vi "GetConnectionStatus.vi"(8 "error in (no error)":errorcluster, 11 "object in":refnum<class "DIO_Channel.lvclass">) -> (0 "error out":errorcluster, 2 "Connected?":bool, 3 "object out":refnum<class "DIO_Channel.lvclass">)   [LabVIEW 2021, in "Simulator-Channel.lvlib" / "DIO_Channel.lvclass"]
uses:
  DIO_Channel.lvclass
  <vilib>/ActorFramework/Message Enqueuer/Message Enqueuer.lvclass
  DIO_Channel.lvclass/DIO_Channel.ctl
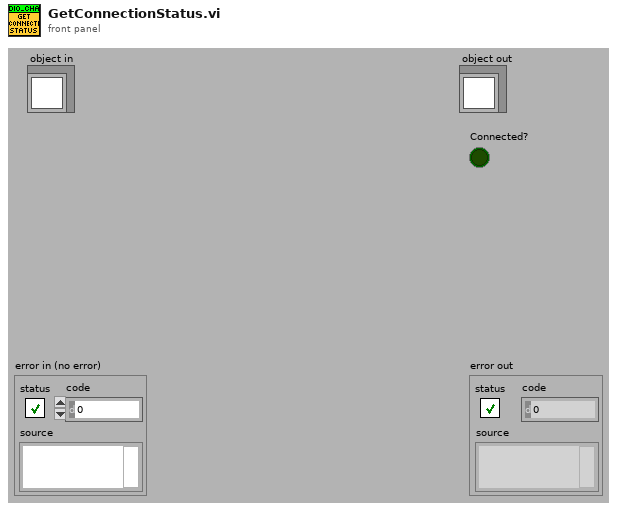
[diagram p1: front panel]
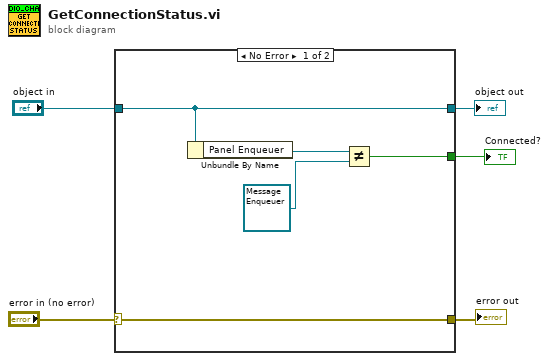
[diagram p0: block diagram]
diagram:
  n1 = case shown="No Error" "error in (no error)" {
    selector: "error in (no error)" -> [w10 w12]
    tunnel: [w10 w12] -> w4
    tunnel: [w9 w11] -> w2
    tunnel: "object in" -> [w9 w11]
    tunnel: [w6 _] -> w1
    frame No Error {
      n2 = Unbundle By Name(w9) -> ("Panel Enqueuer"=w8:refnum<class "Message Enqueuer.lvclass">)
      n3 = Not Equal?(x=w8, y=refnum<class "Message Enqueuer.lvclass"> refnum ("Panel Enqueuer")) -> (x != y?=w6:bool)
    }
    frame Error {
    }
  }
  "error out" <- w4
  "object out" <- w2
  "Connected?" <- w1
